vi "Repeat Until Count.vi"(8 "On Count Status":T1, 9 "Count":i32, 10 "Finish On":T2, 11 "Node In":refnum<class "bt_Node.lvclass">) -> (3 "Node Out":refnum<class "bt_Node.lvclass">)   [LabVIEW 2021]
uses:
  Support/Nodes/Decorators/Repeat Until Count/bt_Repeat Until Count.lvclass
  C:/Users/Tim/Documents/GitHub/LV_Behaviour_Tree/Source/Support/Nodes/abs_Node/bt_Node.lvclass
  Support/Nodes/abs_Node/bt_Node.lvclass
  Support/Nodes/Decorators/Repeater/Support/Finish On - Type.ctl
  Support/Nodes/Decorators/Repeater/bt_Repeater.lvclass
  Support/Nodes/Decorators/Repeat Until Count/Support/On Count Status - Type.ctl
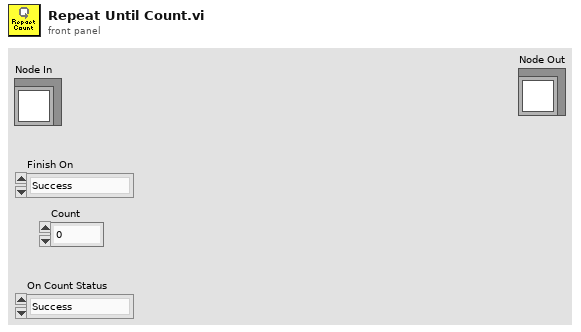
[diagram p1: front panel]
types:
  T1 = typedef "BT.lvlib/bt_Repeat Until Count.lvclass/On Count Status - Type.ctl" = enum16{"Success", "Failure"}
  T2 = typedef "BT.lvlib/bt_Repeater.lvclass/Finish On - Type.ctl" = enum16{"Success", "Failure", "Never"}
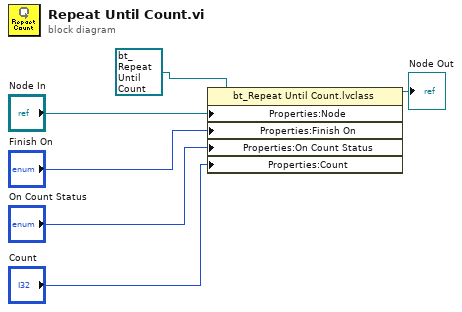
[diagram p0: block diagram]
diagram:
  n1 = property class="bt_Repeat Until Count.lvclass"(reference=refnum<class "bt_Repeat Until Count.lvclass"> refnum ("BT.lvlib:Repeat Until Count.lvclass"), "Properties:Node"="Node In", "Properties:Finish On"="Finish On", "Properties:On Count Status"="On Count Status", "Properties:Count"="Count") -> (reference out=→"Node Out":refnum<class "bt_Repeat Until Count.lvclass">)  [unwired: 1 in, 1 out]
